vi "VIH Project Tree - Item Type to-from Icon Index.vi"(7 "Not found":bool, 11 "Item Type":T1) -> (3 "Icon Index out":i32)   [LabVIEW 2014]
doc: "::: VI Helpeks :::\nCopyright (c) 2000-2026 Konstantin Shifershteyn. All rights reserved."
uses:
  VIH Project Tree Typedef - Tree Item Type.ctl
panel:
  out "Item Type out":T1
  in  "Icon Index":i32
  # "VI Helpeks\nCopyright (c) 2012-2026 Konstantin Shifershteyn"
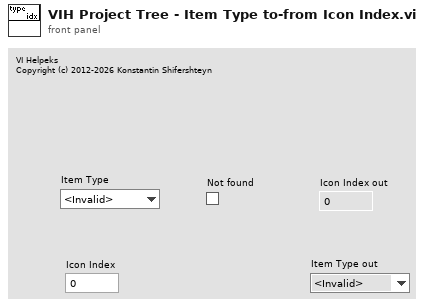
[diagram p1: front panel]
types:
  T1 = typedef "VIH Project Tree Typedef - Tree Item Type.ctl" = enum32{"<Invalid>", "Project", "Proj Files", "Proj Rules", "File Group", "Rule Group", "Any File", "LV Func", ".mnu", ".mnu (dyn)", ".vi", ".vi (dyn)", ".vit", ".vit (dyn)", ".ctl", ".ctl (dyn)", ".ctt", ".ctt (dyn)", "polyVI", "polyVI (dyn)", "expVI", "expVI (dyn)", "HTML", "PolyVI Inst"}
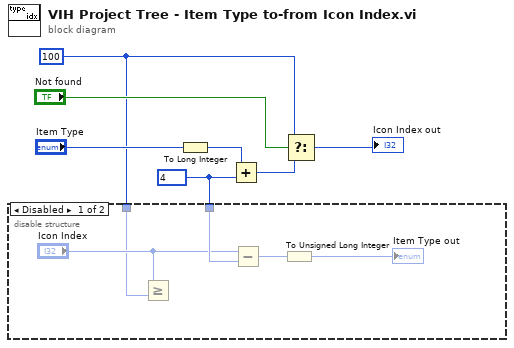
[diagram p0: block diagram]
diagram:
  w1 = 100 ("t")
  w5 = 4
  n1 = disable-structure shown="Disabled" {
    disable-tunnel: w5 -> [w12 _]
    disable-tunnel: w1 -> [w8 _]
    frame Disabled {
      n2 = Greater Or Equal?(x="Icon Index", y=w8) -> ()  [unwired: 1 out]
      n3 = Subtract(x="Icon Index", y=w12) -> (x-y=w11:i32)
      n4 = To Unsigned Long Integer(number=w11) -> (unsigned 32bit integer=→"Item Type out":u32)
    }
    frame Enabled {
    }
  }
  n5 = To Long Integer(number="Item Type") -> (32bit integer=w6:i32)
  n6 = Add(x=w6, y=w5) -> (x+y=w4:i32)
  n7 = Select(t=w1, s="Not found", f=w4) -> (s? t:f=→"Icon Index out":i32)
